vi "Check Start or Stop.vi"(8 "error in (no error)":errorcluster, 9 "Target (All)":string, 10 "Log Group (All)":T1, 11 "GroupLoggingControl in":refnum<class "GroupLoggingControl.lvclass">) -> (0 "error out":errorcluster, 2 "Logging":bool, 3 "GroupLoggingControl out":refnum<class "GroupLoggingControl.lvclass">)   [LabVIEW 2020, in "VolatusGUIElements.lvlib" / "GroupLoggingControl.lvclass"]
uses:
  GroupLoggingControl.lvclass
  Log Group.ctl
  Log Group Status.ctl
  Command Info.ctl
  GroupLoggingControl.lvclass/GroupLoggingControl.ctl
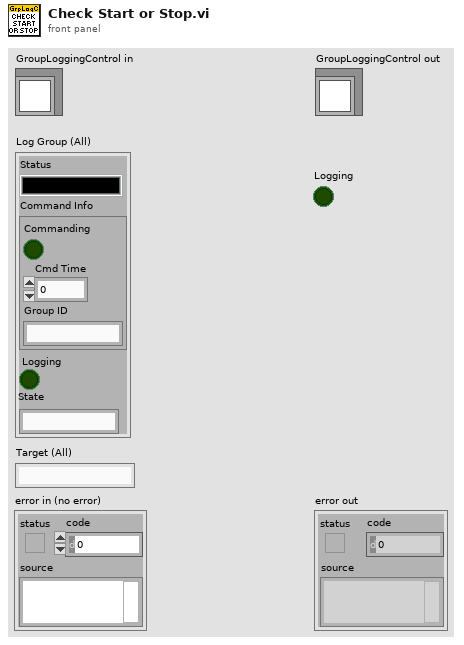
[diagram p1: front panel]
types:
  T1 = typedef "VolatusGUIElements.lvlib/GroupLoggingControl.lvclass/Log Group.ctl" = cluster{"Status":T2, "Command Info":T3, "Logging":bool, "State":string}
  T2 = typedef "VolatusGUIElements.lvlib/GroupLoggingControl.lvclass/Log Group Status.ctl" = cluster{"Group":string, "Group Color":u32, "Button":bool}
  T3 = typedef "VolatusGUIElements.lvlib/GroupLoggingControl.lvclass/Command Info.ctl" = cluster{"Commanding":bool, "Cmd Time":dbl, "Group ID":string}
  T4 = typedef "VolatusGUIElements.lvlib/GroupLoggingControl.lvclass/Status.ctl" = cluster{"Groups":T1[], "Targets":T5[]}
  T5 = typedef "VolatusGUIElements.lvlib/GroupLoggingControl.lvclass/Target Info.ctl" = cluster{"Node":string, "Node Color":u32, "Groups":T1[]}
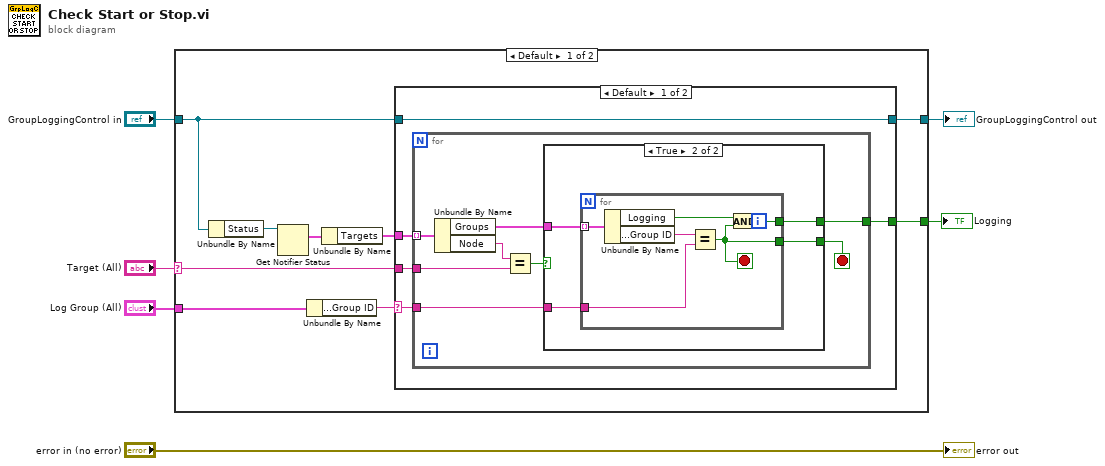
[diagram p0: block diagram]
diagram:
  n1 = case shown="Default" "Target (All)" {
    selector: "Target (All)" -> [w12 _]
    tunnel: "GroupLoggingControl in" -> [w9 w40]
    tunnel: "Log Group (All)" -> [w15 _]
    tunnel: [w11 w40] -> w2
    tunnel: [w10 _] -> w1
    frame Default {
      n2 = Unbundle By Name(w9) -> ("Status"=w8:refnum<notifier>)
      n3 = Get Notifier Status(notifier=w8) -> (current notification=w7:T4)  [unwired: 1 in, 4 out]
      n4 = Unbundle By Name(w15) -> ("Command Info.Group ID"=w14:string)
      n5 = Unbundle By Name(w7) -> ("Targets"=w13:T5[])
      n6 = case shown="Default" w14 {
        selector: w14 -> [w17 _]
        tunnel: w9 -> [w20 w39]
        tunnel: w13 -> [w19 _]
        tunnel: w12 -> [w18 _]
        tunnel: [w20 w39] -> w11
        tunnel: [w16 _] -> w10
        frame Default {
          n7 = for {
            tunnel: w19 -> [w28] mode=indexing
            tunnel: w18 -> [w27]
            tunnel: w17 -> [w23]
            tunnel: [w22] -> w16
            stop <- w21 stop-if-true
            n8 = Unbundle By Name(w28) -> ("Groups"=w24:T1[], "Node"=w26:string)
            n9 = Equal?(x=w26, y=w27) -> (x = y?=w25:bool)
            n10 = case shown="True" w25 {
              tunnel: w24 -> [_ w32]
              tunnel: w23 -> [_ w31]
              tunnel: [_ w30] -> w22
              tunnel: [_ w29] -> w21
              frame False {
              }
              frame True {
                n11 = for {
                  tunnel: w32 -> [w38] mode=indexing
                  tunnel: w31 -> [w36]
                  tunnel: [w34] -> w30
                  tunnel: [w33] -> w29
                  stop <- w33 stop-if-true
                  n12 = Unbundle By Name(w38) -> ("Logging"=w35:bool, "Command Info.Group ID"=w37:string)
                  n13 = Equal?(x=w37, y=w36) -> (x = y?=w33:bool)
                  n14 = And(x=w35, y=w33) -> (x .and. y?=w34:bool)
                }
              }
            }
          }
        }
        frame "True" {
        }
      }
    }
    frame "" {
      # "All Targets"
    }
  }
  "GroupLoggingControl out" <- w2
  "Logging" <- w1
  "error out" <- "error in (no error)"
